vi "Ballard Multichannel Tx and RX PARAM Constants.vi"(1 "Transfer Type":enum16{"Acyclic", "Scheduled"}(ring)) -> (0 "Parameters (3D Array)":i32[][][](array[numeric]))   [LabVIEW 2020]
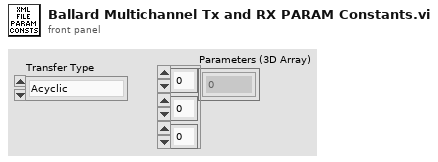
[diagram p1: front panel]
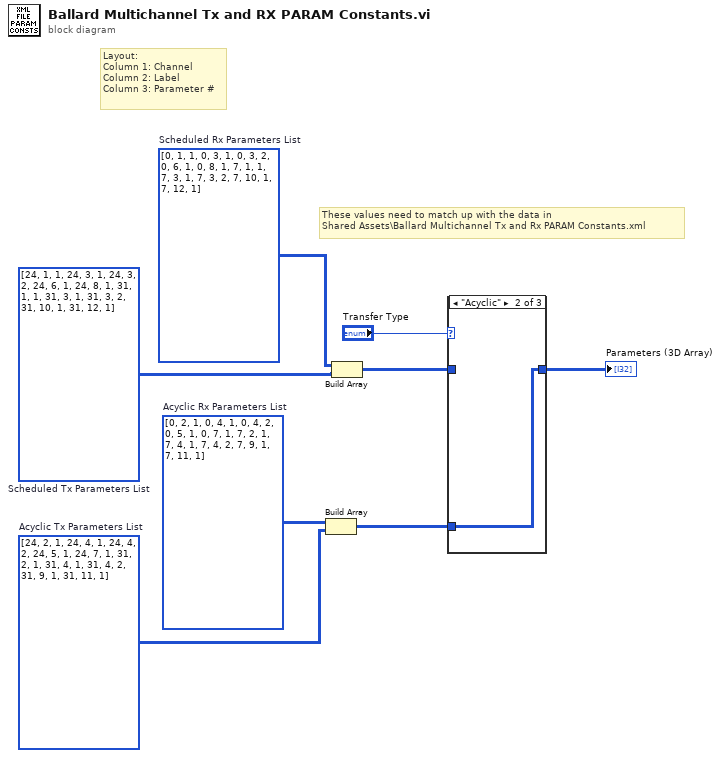
[diagram p0: block diagram]
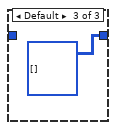
[diagram p3: hidden frame]
diagram:
  w2 = i32[][] [[0, 2, 1], [0, 4, 1], [0, 4, 2], [0, 5, 1], [0, 7, 1], [7, 2, 1], [7, 4, 1], [7, 4, 2], [7, 9, 1], [7, 11, 1]]  # Acyclic Rx Parameters List
  w4 = i32[][] [[0, 1, 1], [0, 3, 1], [0, 3, 2], [0, 6, 1], [0, 8, 1], [7, 1, 1], [7, 3, 1], [7, 3, 2], [7, 10, 1], [7, 12, 1]]  # Scheduled Rx Parameters List
  w1 = i32[][] [[24, 2, 1], [24, 4, 1], [24, 4, 2], [24, 5, 1], [24, 7, 1], [31, 2, 1], [31, 4, 1], [31, 4, 2], [31, 9, 1], [31, 11, 1]]  # Acyclic Tx Parameters List
  w3 = i32[][] [[24, 1, 1], [24, 3, 1], [24, 3, 2], [24, 6, 1], [24, 8, 1], [31, 1, 1], [31, 3, 1], [31, 3, 2], [31, 10, 1], [31, 12, 1]]  # Scheduled Tx Parameters List
  # "These values need to match up with the data in\nShared Assets\\Ballard Multichannel Tx and Rx PARAM Constants.xml"
  # "Layout:\nColumn 1: Channel\nColumn 2: Label\nColumn 3: Parameter #"
  n1 = Build Array(w2, w1) -> (w5:i32[][][])
  n2 = Build Array(w4, w3) -> (w6:i32[][][])
  n3 = case shown="\"Acyclic\"" "Transfer Type" {
    tunnel: [w9 w10 i32[][][] [] ("Parameters (3D Array)")] -> w7
    tunnel: w6 -> [w9 _ _]
    tunnel: w5 -> [_ w10 _]
    frame "Scheduled" {
    }
    frame "Acyclic" {
    }
    frame Default {
    }
  }
  "Parameters (3D Array)" <- w7
